vi "Measurement UI.vi"() -> ()   [LabVIEW 2025, in "Digital Pattern Sequencer UI.lvlib"]
uses:
  Digital Pattern Sequencer UI.lvlib
  <vilib>/xml/Load XML String.vi
  <vilib>/xml/Close Reference(Node).vi
  <vilib>/xml/NI_XML.lvlib
  <resource>/objmgr/DOMUserDefRef.rc
panel:
  in  "Apply TDR?":bool caption="Apply TDR? (If Provided)"
  in  "DUT Bring Up":string(combo) caption="DUT Bring Up* (Blank If Not Required)"
  in  "Tab Control":enum32{"Pattern List", "Results", "Hidden"}(tab)
  out "Total Pattern to Burst":dbl
  in  "Pattern":string(combo)
  in  "Current Measurement Pin":string(combo) caption="Current Measurement Pin\n(Blank If Not Required)"
  in  "Add to List":bool
  in  "Pattern List":T1(array[cluster])
  out "Results":string
  out "All Pass?":bool
  in  "List-Current Measurement Pins":string[](array[string])
  in  "List-Patterns":string[](array[string])
  in  "Reload Project":bool
  in  "Site":i32
  in  "DPE Project File Path":path
  # "* Run power sequence and bring-up pattern only"
  # "This list can be edited. Right click to see more options such as remove or copy item.\nNOTE: Pattern may fail to complete/execute if register, flag, event signal, or jump triggers is used."
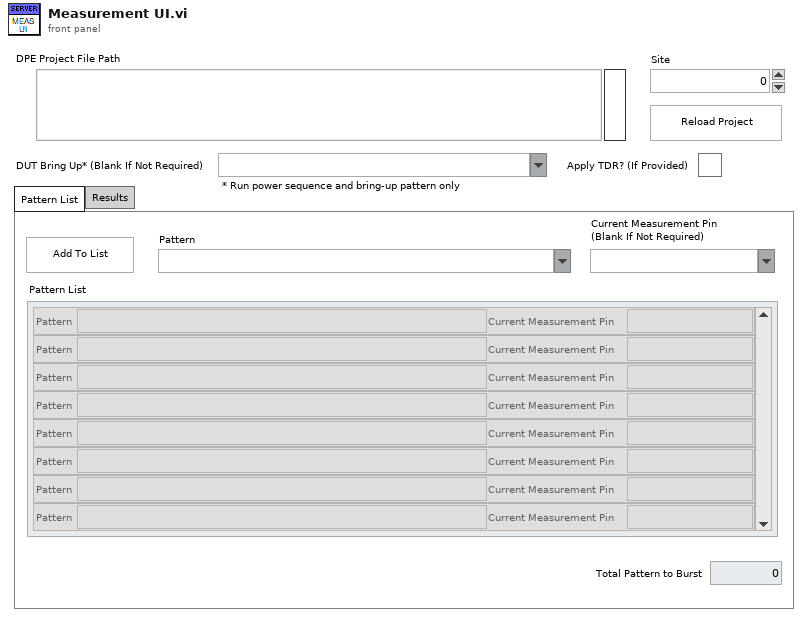
[diagram p1: front panel]
types:
  T1 = cluster{"Pattern":string, "Current Measurement Pin":string}[]
  T2 = cluster{"Pattern":string, "Current Measurement Pin":string}
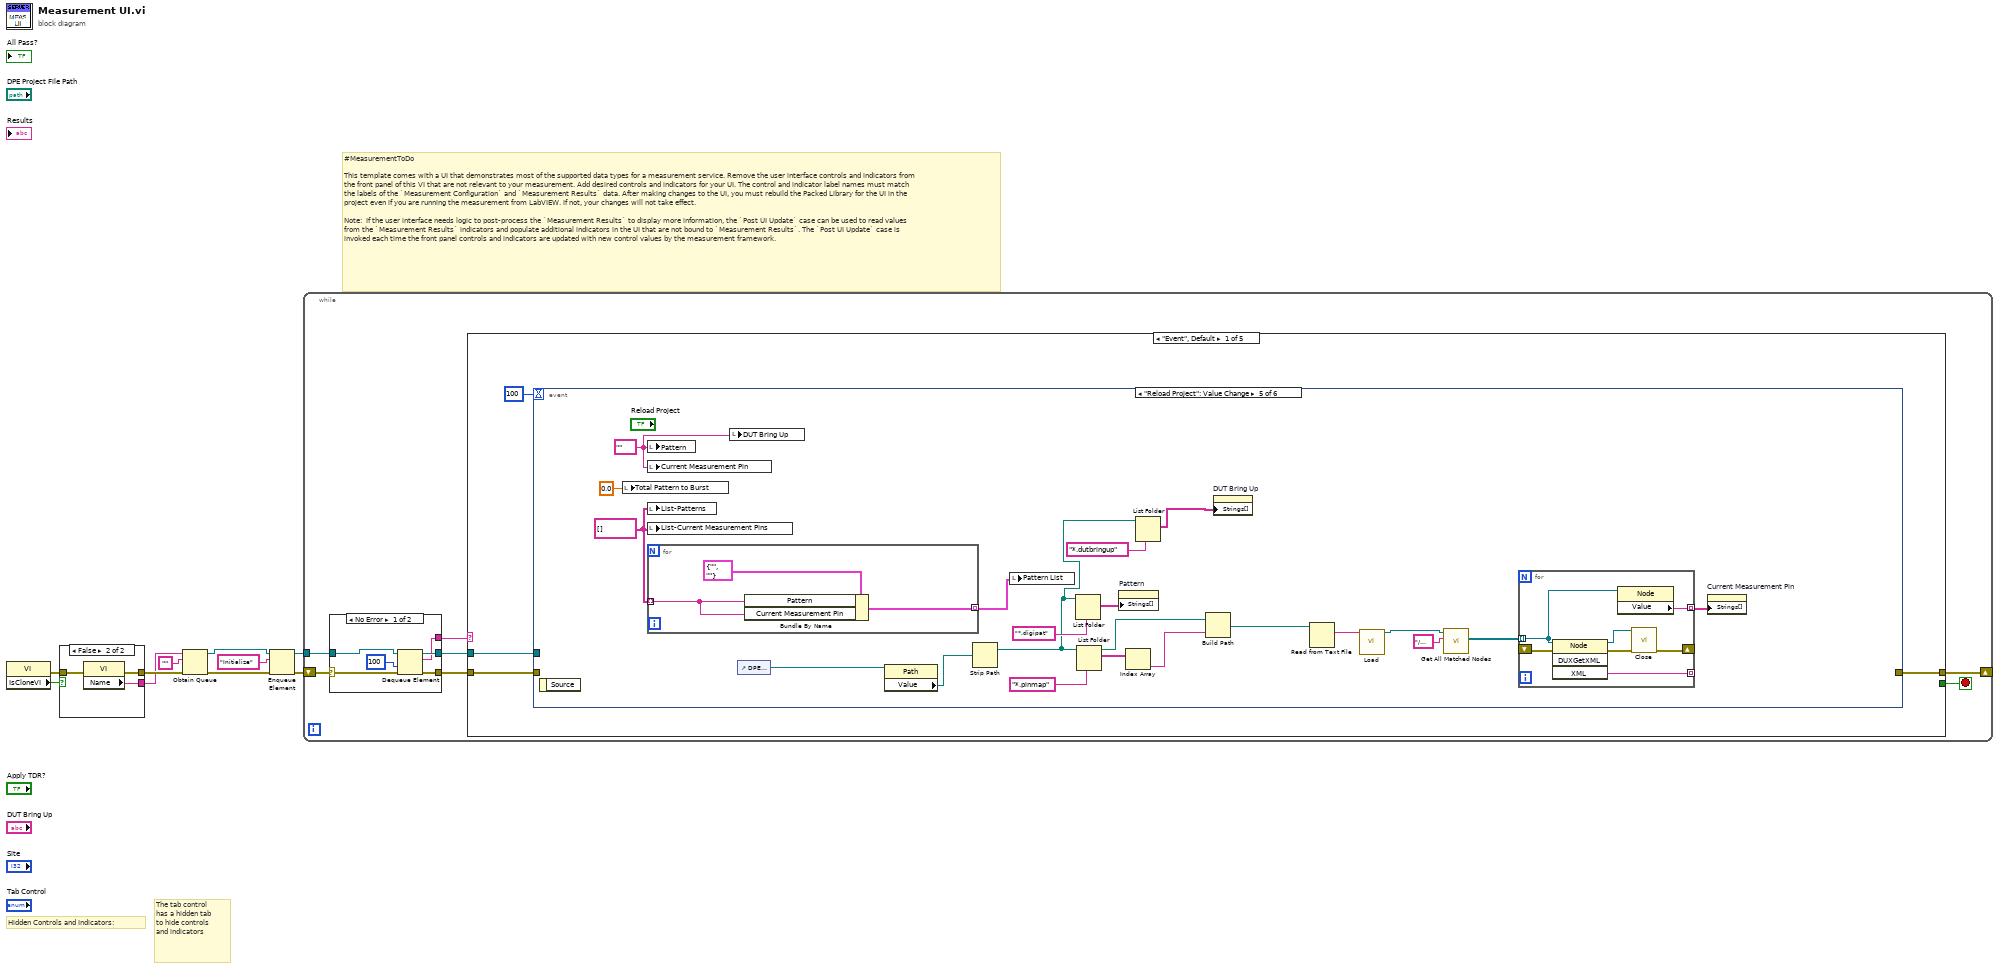
[diagram p0: block diagram]
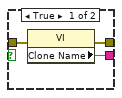
[diagram p2: hidden frame]
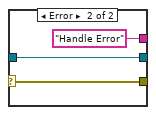
[diagram p3: hidden frame]
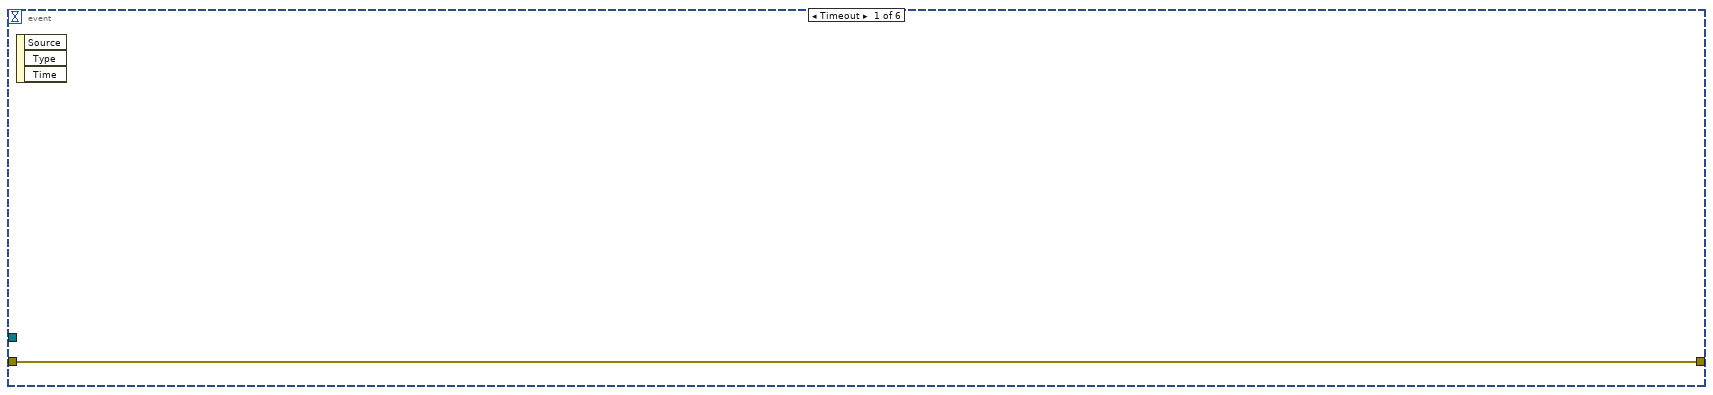
[diagram p4: hidden frame]
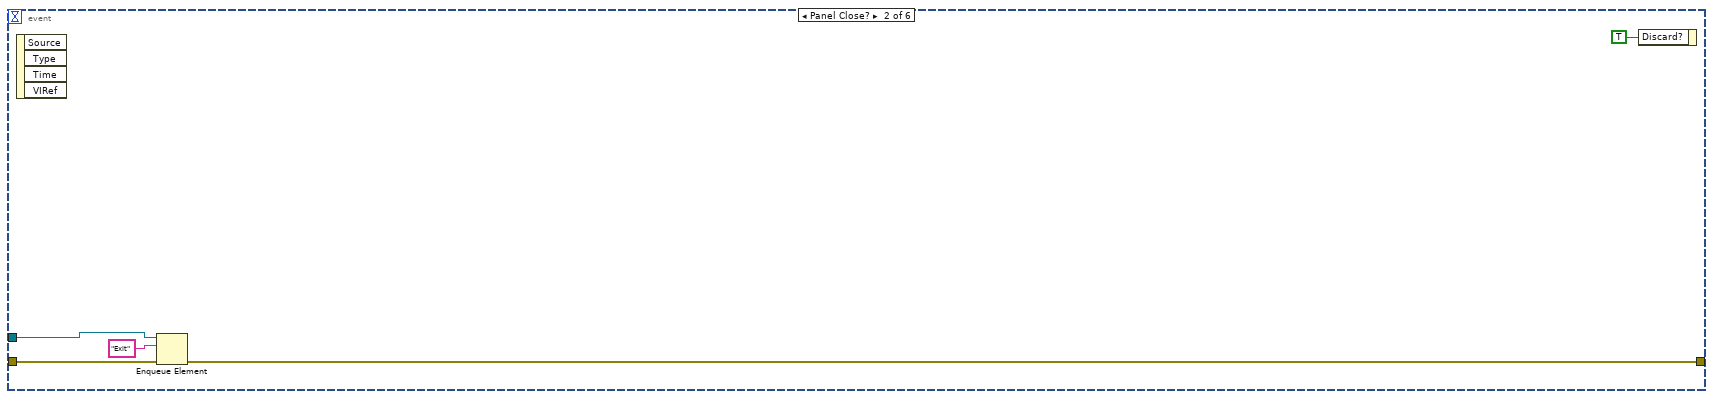
[diagram p5: hidden frame]
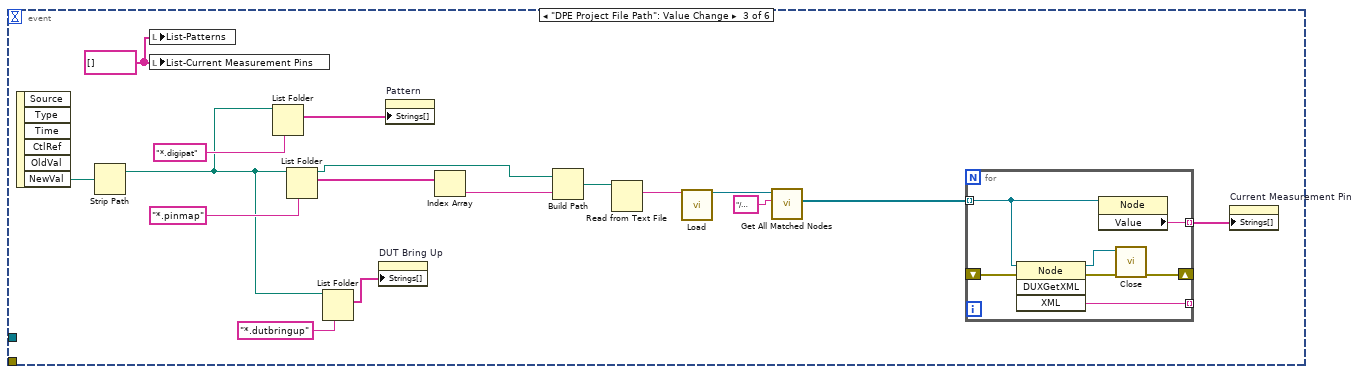
[diagram p6: hidden frame]
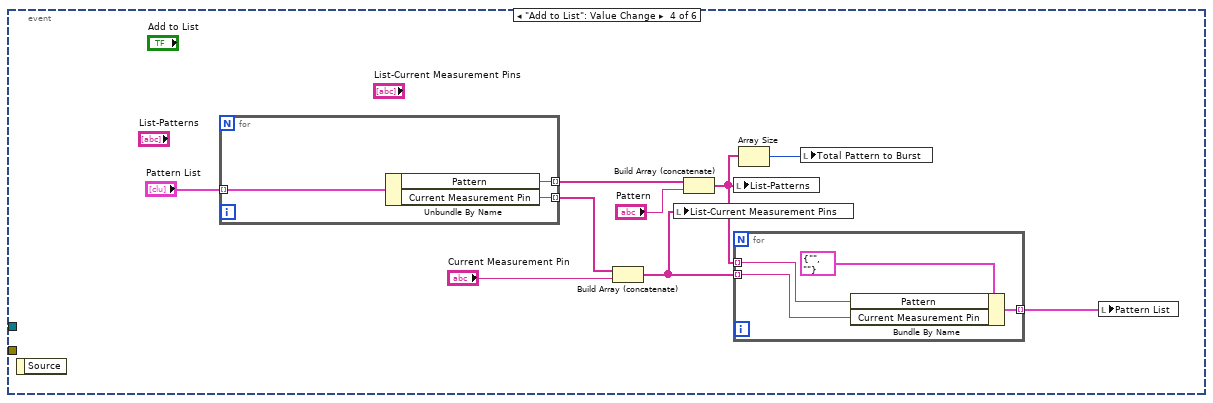
[diagram p7: hidden frame]
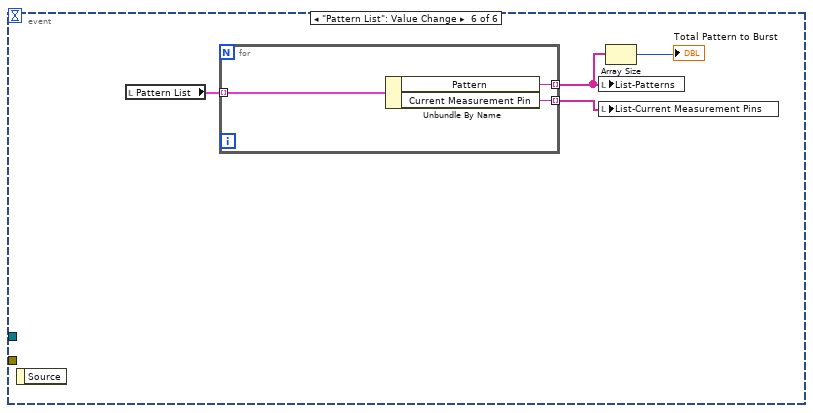
[diagram p8: hidden frame]
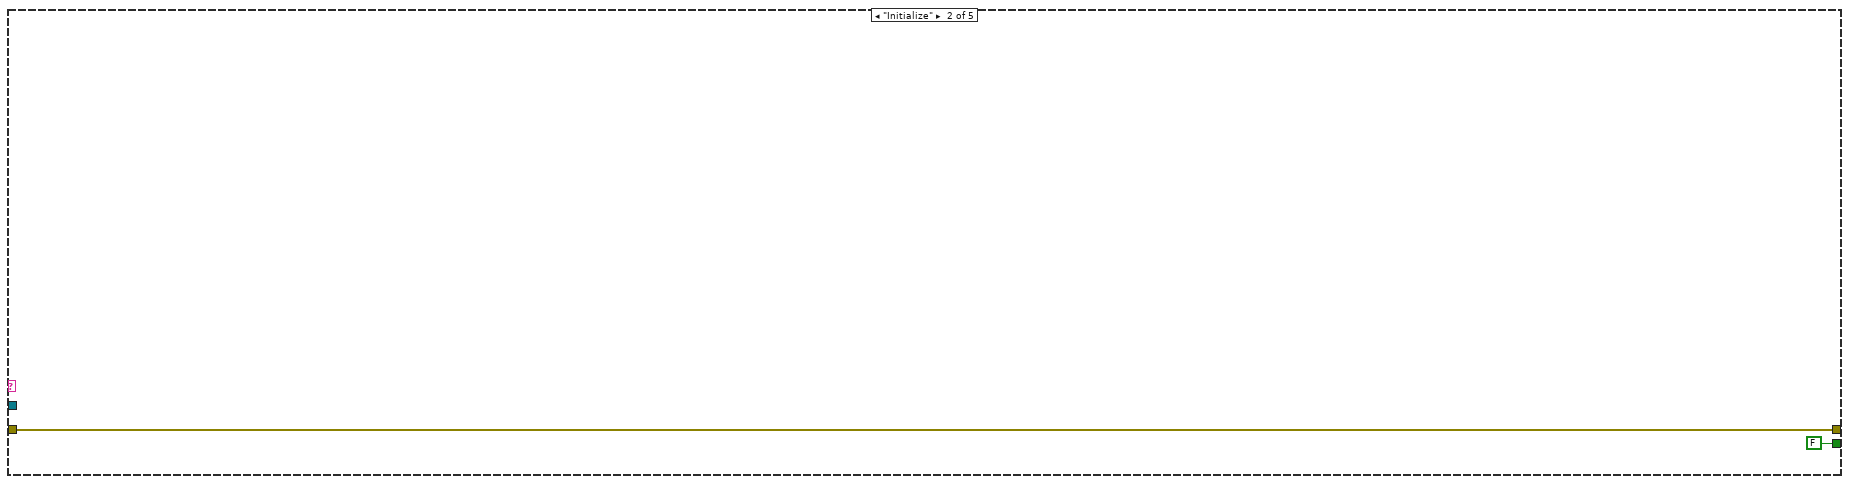
[diagram p9: hidden frame]
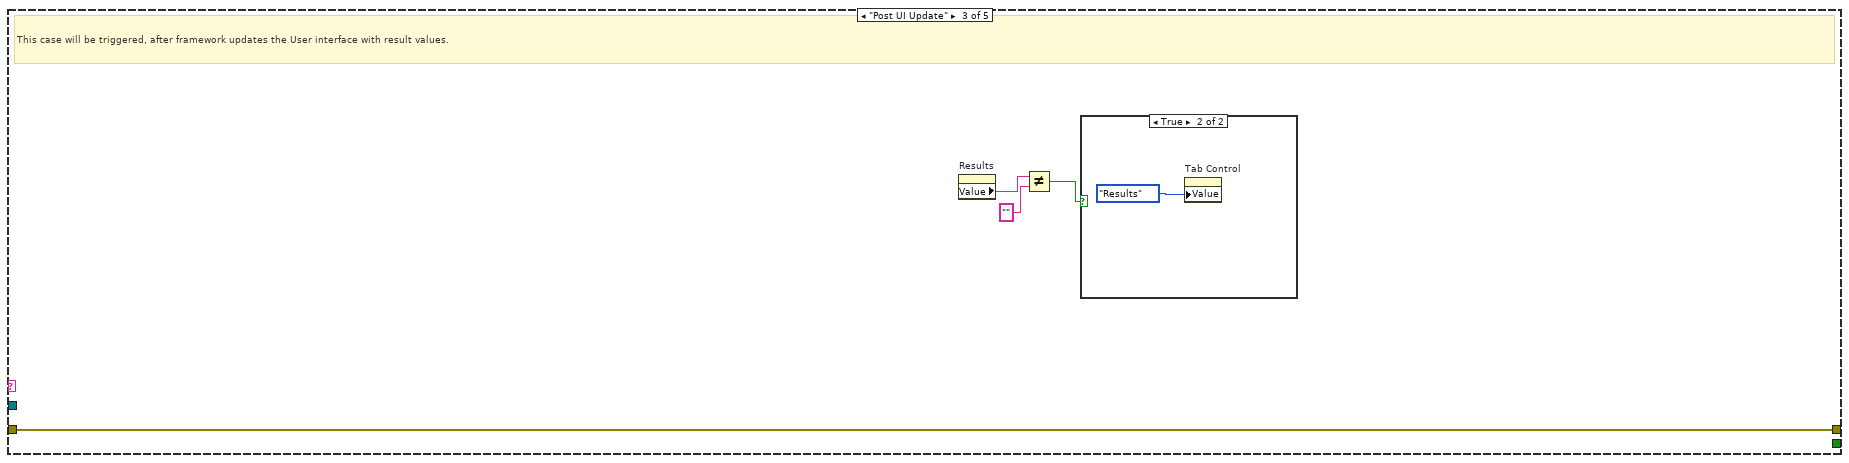
[diagram p10: hidden frame]
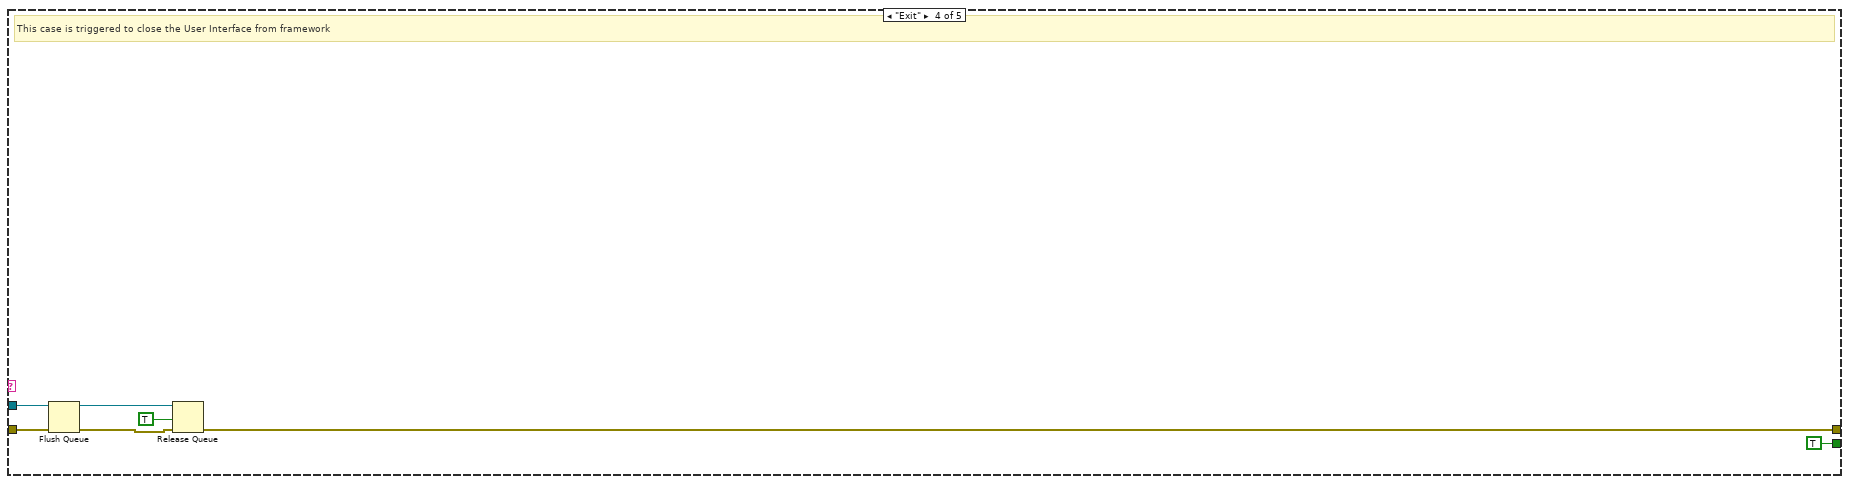
[diagram p12: hidden frame]
diagram:
  # "Hidden Controls and Indicators:"
  # "The tab control has a hidden tab to hide controls and indicators"
  # "#MeasurementToDo  \n\nThis template comes with a UI that demonstrates most of the supported data types for a measurement service. Remove the user interface controls and indicators from the front panel of this VI that are not relevant to your measurement. Add desired controls and indicators for your UI. The control and indicator label names must match the labels of the `Measurement Configuration` and `Measurement Results` data. After making changes to the UI, you must rebuild the Packed Library for the UI in the project even if you are running the measurement from LabVIEW. If not, your changes will not take effect.\n\nNote:  If the user interface needs logic to post-process the `Measurement Results` to display more information, the `Post UI Update` case can be used to read values from the `Measurement Results` indicators and populate additional indicators in the UI that are not bound to `Measurement Results`. The `Post UI Update` case is invoked each time the front panel controls and indicators are updated with new control values by the measurement framework."
  n1 = property class="VI"() -> (error out=w1:errorcluster, "IsCloneVI"=w2:bool)  [unwired: 2 in, 1 out]
  n2 = case shown="False" w2 {
    tunnel: [w13 w16] -> w10
    tunnel: [w12 w15] -> w9
    tunnel: w1 -> [w11 w14]
    frame True {
      n3 = property class="VI"(error in=w11) -> (error out=w13:errorcluster, "Clone Name"=w12:string)  [unwired: 1 in, 1 out]
    }
    frame False {
      n4 = property class="VI"(error in=w14) -> (error out=w16:errorcluster, "Name"=w15:string)  [unwired: 1 in, 1 out]
    }
  }
  n5 = Obtain Queue(name (unnamed)=w9, element data type="", error in (no error)=w10) -> (queue out=w6:refnum<queue>, error out=w8:errorcluster)  [unwired: 2 in, 1 out]
  n6 = Enqueue Element(queue=w6, element="Initialize", error in (no error)=w8) -> (queue out=w5:refnum<queue>, error out=w7:errorcluster)  [unwired: 1 in, 1 out]
  n7 = while {
    shift-right: [w18] -> _
    shift-left: w7 -> [w23]
    tunnel: w5 -> [w21]
    stop <- w17 stop-if-true
    n8 = case shown="No Error" w23 {
      selector: w23 -> [w29 w32]
      tunnel: [w28 w32] -> w22
      tunnel: w21 -> [w27 w31]
      tunnel: [w26 w31] -> w20
      tunnel: [w25 "Handle Error"] -> w19
      frame No Error {
        n9 = Dequeue Element(queue=w27, timeout in ms (-1)=100, error in (no error)=w29) -> (queue out=w26:refnum<queue>, element=w25:string, error out=w28:errorcluster)  [unwired: 1 out]
      }
      frame Error {
      }
    }
    n10 = case shown="\"Event\", Default" w19 {
      tunnel: w22 -> [w35 w122 w126 w134 w135]
      tunnel: w20 -> [w33 _ _ w132 _]
      tunnel: [w36 w122 w126 w129 w135] -> w18
      tunnel: [_ FALSE _ TRUE _] -> w17
      frame "Event", Default {
        n11 = event shown="[4] \"Reload Project\": Value Change" {
          selector: _ -> [_ _ _ _ _ _]
          dyn-events: _ -> [_ _ _ _ _ _]
          timeout: 100 -> [_ _ _ _ _ _]
          tunnel: [w37 w40 _ _ _ _] -> w36
          tunnel: w35 -> [w37 w41 _ _ _ _]
          tunnel: w33 -> [_ w39 _ _ _ _]
          event Timeout {
            n12 = event-data() -> ()  [unwired: 1 in, 3 out]
          }
          event Panel Close? {
            n13 = event-data() -> ()  [unwired: 1 in, 4 out]
            n14 = Enqueue Element(queue=w39, element="Exit", error in (no error)=w41) -> (error out=w40:errorcluster)  [unwired: 1 in, 2 out]
            n15 = event-data("Discard?"=TRUE) -> ()  [unwired: 1 in, 1 out]
          }
          event "DPE Project File Path": Value Change {
            w47 = string[] []
            n16 = event-data() -> ("NewVal"=w57:path)  [unwired: 1 in, 5 out]
            n17 = Strip Path(path=w57) -> (stripped path=w45:path)  [unwired: 1 out]
            n18 = local write "List-Patterns"(w47) -> ()
            n19 = local write "List-Current Measurement Pins"(w47) -> ()
            n20 = List Folder(path=w45, pattern="*.digipat") -> (filenames=w58:string[])  [unwired: 2 in, 3 out]
            n21 = List Folder(path=w45, pattern="*.pinmap") -> (path out=w55:path, filenames=w54:string[])  [unwired: 2 in, 2 out]
            n22 = List Folder(path=w45, pattern="*.dutbringup") -> (filenames=w43:string[])  [unwired: 2 in, 3 out]
            n23 = property on="DUT Bring Up" class="CmbBox"("Strings[]"=w43) -> ()  [unwired: 2 in, 2 out]
            n24 = property on="Pattern" class="CmbBox"("Strings[]"=w58) -> ()  [unwired: 2 in, 2 out]
            n25 = Index Array(array=w54) -> (element=w53:string)  [unwired: 1 in]
            n26 = Build Path(base path=w55, name or relative path=w53) -> (appended path=w52:path)
            n27 = Read from Text File(file (use dialog)=w52) -> (text=w51:string)  [unwired: 3 in, 3 out]
            n28 = call-poly <vilib>:"Load.vi"("XML string"=w51) -> ("DOM document out"=w50:refnum<k20>)  [unwired: 12 in, 2 out]
            n29 = call <vilib>:"Get All Matched Nodes.vi"("XPath expression"="/PinMap/Connections/Connection/@pin", "node in"=w50) -> ("node result array"=w48:refnum<k20>[])  [unwired: 1 in, 8 out]
            n30 = for {
              tunnel: w48 -> [w61] mode=indexing
              shift-right: [w64] -> _
              shift-left: _ -> [w63]
              tunnel: [w62] -> _ mode=indexing
              tunnel: [w60] -> w46 mode=indexing
              n31 = invoke on="Invoke Node" class="Node" method="DUXGetXML"(reference=w61, error in=w63) -> (reference out=w65:refnum<k20>, error out=w66:errorcluster, "XML"=w62:string)  [unwired: 2 in, 1 out]
              n32 = property class="Node"(reference=w61) -> ("Value"=w60:string)  [unwired: 1 in, 2 out]
              n33 = call-poly <vilib>:"Close.vi"("error in (no error)"=w66, "node"=w65) -> ("error out"=w64:errorcluster)  [unwired: 7 out]
            }
            n34 = property on="Current Measurement Pin" class="CmbBox"("Strings[]"=w46) -> ()  [unwired: 2 in, 2 out]
          }
          event "Add to List": Value Change {
            n35 = event-data() -> ()  [unwired: 1 in, 1 out]
            n36 = for {
              tunnel: "Pattern List" -> [w78] mode=indexing
              tunnel: [w77] -> w70 mode=indexing
              tunnel: [w76] -> w69 mode=indexing
              n37 = Unbundle By Name(w78) -> ("Pattern"=w77:string, "Current Measurement Pin"=w76:string)
            }
            n38 = Build Array (concatenate)(w69, "Current Measurement Pin") -> (w67:string[])
            n39 = local write "List-Current Measurement Pins"(w67) -> ()
            n40 = Build Array (concatenate)(w70, "Pattern") -> (w68:string[])
            n41 = local write "List-Patterns"(w68) -> ()
            n42 = for {
              tunnel: w68 -> [w81] mode=indexing
              tunnel: w67 -> [w80] mode=indexing
              tunnel: [w79] -> w72 mode=indexing
              n43 = Bundle By Name(cluster=T2 {"Pattern"="", "Current Measurement Pin"=""} ("Pattern List"), "Pattern"=w81, "Current Measurement Pin"=w80) -> (w79:T2)
            }
            n44 = Array Size(array=w68) -> (size(s)=w73:i32)
            n45 = local write "Total Pattern to Burst"(w73) -> ()
            n46 = local write "Pattern List"(w72) -> ()
          }
          event "Reload Project": Value Change {
            w86 = "" ("Pattern")
            w87 = string[] []
            n47 = event-data() -> ()  [unwired: 1 in, 1 out]
            n48 = local write "Total Pattern to Burst"(0.0 ("Total Pattern to Burst")) -> ()
            n49 = local write "Pattern"(w86) -> ()
            n50 = local write "Current Measurement Pin"(w86) -> ()
            n51 = local write "List-Patterns"(w87) -> ()
            n52 = local write "List-Current Measurement Pins"(w87) -> ()
            n53 = for {
              tunnel: [w105] -> w88 mode=indexing
              tunnel: w87 -> [w104] mode=indexing
              n54 = Bundle By Name(cluster=T2 {"Pattern"="", "Current Measurement Pin"=""} ("Pattern List"), "Pattern"=w104, "Current Measurement Pin"=w104) -> (w105:T2)
            }
            n55 = local write "DUT Bring Up"(w86) -> ()
            n56 = control-ref of="DPE Project File Path"() -> (w102:refnum<vi>)
            n57 = property class="Path"(reference=w102) -> ("Value"=w101:path)  [unwired: 1 in, 2 out]
            n58 = Strip Path(path=w101) -> (stripped path=w84:path)  [unwired: 1 out]
            n59 = local write "Pattern List"(w88) -> ()
            n60 = List Folder(path=w84, pattern="*.digipat") -> (filenames=w100:string[])  [unwired: 2 in, 3 out]
            n61 = List Folder(path=w84, pattern="*.pinmap") -> (path out=w98:path, filenames=w97:string[])  [unwired: 2 in, 2 out]
            n62 = property on="Pattern" class="CmbBox"("Strings[]"=w100) -> ()  [unwired: 2 in, 2 out]
            n63 = Index Array(array=w97) -> (element=w96:string)  [unwired: 1 in]
            n64 = List Folder(path=w84, pattern="*.dutbringup") -> (filenames=w83:string[])  [unwired: 2 in, 3 out]
            n65 = Build Path(base path=w98, name or relative path=w96) -> (appended path=w95:path)
            n66 = property on="DUT Bring Up" class="CmbBox"("Strings[]"=w83) -> ()  [unwired: 2 in, 2 out]
            n67 = Read from Text File(file (use dialog)=w95) -> (text=w94:string)  [unwired: 3 in, 3 out]
            n68 = call-poly <vilib>:"Load.vi"("XML string"=w94) -> ("DOM document out"=w93:refnum<k20>)  [unwired: 12 in, 2 out]
            n69 = call <vilib>:"Get All Matched Nodes.vi"("XPath expression"="/PinMap/Connections/Connection/@pin", "node in"=w93) -> ("node result array"=w91:refnum<k20>[])  [unwired: 1 in, 8 out]
            n70 = for {
              tunnel: w91 -> [w108] mode=indexing
              shift-right: [w111] -> _
              shift-left: _ -> [w110]
              tunnel: [w109] -> _ mode=indexing
              tunnel: [w107] -> w89 mode=indexing
              n71 = invoke on="Invoke Node" class="Node" method="DUXGetXML"(reference=w108, error in=w110) -> (reference out=w112:refnum<k20>, error out=w113:errorcluster, "XML"=w109:string)  [unwired: 2 in, 1 out]
              n72 = property class="Node"(reference=w108) -> ("Value"=w107:string)  [unwired: 1 in, 2 out]
              n73 = call-poly <vilib>:"Close.vi"("error in (no error)"=w113, "node"=w112) -> ("error out"=w111:errorcluster)  [unwired: 7 out]
            }
            n74 = property on="Current Measurement Pin" class="CmbBox"("Strings[]"=w89) -> ()  [unwired: 2 in, 2 out]
          }
          event "Pattern List": Value Change {
            n75 = event-data() -> ()  [unwired: 1 in, 1 out]
            n76 = local read "Pattern List"() -> (w116:T1)
            n77 = for {
              tunnel: w116 -> [w120] mode=indexing
              tunnel: [w119] -> w114 mode=indexing
              tunnel: [w118] -> w115 mode=indexing
              n78 = Unbundle By Name(w120) -> ("Pattern"=w119:string, "Current Measurement Pin"=w118:string)
            }
            n79 = local write "List-Patterns"(w114) -> ()
            n80 = local write "List-Current Measurement Pins"(w115) -> ()
            n81 = Array Size(array=w114) -> (size(s)=→"Total Pattern to Burst":i32)
          }
        }
      }
      frame "Initialize" {
      }
      frame "Post UI Update" {
        # "This case will be triggered, after framework updates the User interface with result values."
        n82 = property on="Results" class="Str"() -> ("Value"=w125:string)  [unwired: 2 in, 2 out]
        n83 = Not Equal?(x=w125, y="") -> (x != y?=w123:bool)
        n84 = case shown="True" w123 {
          frame False {
          }
          frame True {
            n85 = property on="Tab Control" class="TabCtl (strict)"("Value"=enum32{"Pattern List", "Results", "Hidden"}."Results" ("Tab Control")) -> ()  [unwired: 2 in, 2 out]
          }
        }
      }
      frame "Exit" {
        # "This case is triggered to close the User Interface from framework"
        n86 = Flush Queue(queue=w132, error in (no error)=w134) -> (queue out=w131:refnum<queue>, error out=w130:errorcluster)  [unwired: 1 out]
        n87 = Release Queue(queue=w131, force destroy? (F)=TRUE, error in (no error)=w130) -> (error out=w129:errorcluster)  [unwired: 2 out]
      }
      frame "Handle Error" {
      }
    }
  }
